vi "MecaOdometry_Update.vi"(9 "WheelPosition":T1 {"RearRight" format="%19.3f"; "RearLeft" format="%19.3f"; "FrontRight" format="%19.3f"; "FrontLeft" format="%19.3f"}, 10 "GyroAngle":T5={"VALUE"=0.0, "COS"=1.0, "SIN"=0.0} {"SIN" format="%13.4f"; "COS" format="%13.4f"; "VALUE" format="%13.4f"}, 11 "in MECA_DRIVE_ODOMETRY":T2={"POSE"={"TRANSLATION"={"X"=0.0, "Y"=0.0}, "ROTATION"={"VALUE"=0.0, "COS"=1.0, "SIN"=0.0}}, "GyroOffset"={"VALUE"=0.0, "COS"=0.0, "SIN"=0.0}, "PreviousAngle"={"VALUE"=0.0, "COS"=0.0, "SIN"=0.0}, "Kinematics"={"FrontLeft"={"X"=0.0, "Y"=0.0}, "FrontRight"={"X"=0.0, "Y"=0.0}, "RearLeft"={"X"=0.0, "Y"=0.0}, "RearRight"={"X"=0.0, "Y"=0.0}, "InverseKinematics"=[[0.0, 1.0, -1.0, 0.0], [0.0, 1.0, 1.0, 0.0], [0.0, 1.0, 1.0, 0.0], [0.0, 1.0, -1.0, 0.0]], "ForwardKinematics"=[[0.0, 1.0, -1.0, 0.0], [0.0, 1.0, 1.0, 0.0], [0.0, 1.0, 1.0, 0.0], [0.0, 1.0, -1.0, 0.0]], "PrevCoR"={"X"=0.0, "Y"=0.0}}, "PreviousWheelPositions"={"FrontLeft"=0.0, "FrontRight"=0.0, "RearLeft"=0.0, "RearRight"=0.0, "P"=FALSE}} {"PreviousWheelPositions"."RearRight" format="%19.3f"; "PreviousWheelPositions"."RearLeft" format="%19.3f"; "PreviousWheelPositions"."FrontRight" format="%19.3f"; "PreviousWheelPositions"."FrontLeft" format="%19.3f"; "Kinematics"."PrevCoR"."Y" format="%14.3f"; "Kinematics"."PrevCoR"."X" format="%14.3f"; "Kinematics"."RearRight"."Y" format="%14.3f"; "Kinematics"."RearRight"."X" format="%14.3f"; "Kinematics"."RearLeft"."Y" format="%14.3f"; "Kinematics"."RearLeft"."X" format="%14.3f"; "Kinematics"."FrontRight"."Y" format="%14.3f"; "Kinematics"."FrontRight"."X" format="%14.3f"; "Kinematics"."FrontLeft"."Y" format="%14.3f"; "Kinematics"."FrontLeft"."X" format="%14.3f"; "PreviousAngle"."SIN" format="%13.4f"; "PreviousAngle"."COS" format="%13.4f"; "PreviousAngle"."VALUE" format="%13.4f"; "GyroOffset"."SIN" format="%13.4f"; "GyroOffset"."COS" format="%13.4f"; "GyroOffset"."VALUE" format="%13.4f"; "POSE"."ROTATION"."SIN" format="%13.4f"; "POSE"."ROTATION"."COS" format="%13.4f"; "POSE"."ROTATION"."VALUE" format="%13.4f"; "POSE"."TRANSLATION"."Y" format="%14.3f"; "POSE"."TRANSLATION"."X" format="%14.3f"}) -> (1 "POSE":T3={"TRANSLATION"={"X"=0.0, "Y"=0.0}, "ROTATION"={"VALUE"=0.0, "COS"=1.0, "SIN"=0.0}} {"ROTATION"."SIN" format="%13.4f"; "ROTATION"."COS" format="%13.4f"; "ROTATION"."VALUE" format="%13.4f"; "TRANSLATION"."Y" format="%14.3f"; "TRANSLATION"."X" format="%14.3f"}, 3 "out MECA_DRIVE_ODOMETRY":T2={"POSE"={"TRANSLATION"={"X"=0.0, "Y"=0.0}, "ROTATION"={"VALUE"=0.0, "COS"=1.0, "SIN"=0.0}}, "GyroOffset"={"VALUE"=0.0, "COS"=0.0, "SIN"=0.0}, "PreviousAngle"={"VALUE"=0.0, "COS"=0.0, "SIN"=0.0}, "Kinematics"={"FrontLeft"={"X"=0.0, "Y"=0.0}, "FrontRight"={"X"=0.0, "Y"=0.0}, "RearLeft"={"X"=0.0, "Y"=0.0}, "RearRight"={"X"=0.0, "Y"=0.0}, "InverseKinematics"=[[0.0, 1.0, -1.0, 0.0], [0.0, 1.0, 1.0, 0.0], [0.0, 1.0, 1.0, 0.0], [0.0, 1.0, -1.0, 0.0]], "ForwardKinematics"=[[0.0, 1.0, -1.0, 0.0], [0.0, 1.0, 1.0, 0.0], [0.0, 1.0, 1.0, 0.0], [0.0, 1.0, -1.0, 0.0]], "PrevCoR"={"X"=0.0, "Y"=0.0}}, "PreviousWheelPositions"={"FrontLeft"=0.0, "FrontRight"=0.0, "RearLeft"=0.0, "RearRight"=0.0, "P"=FALSE}} {"PreviousWheelPositions"."RearRight" format="%19.3f"; "PreviousWheelPositions"."RearLeft" format="%19.3f"; "PreviousWheelPositions"."FrontRight" format="%19.3f"; "PreviousWheelPositions"."FrontLeft" format="%19.3f"; "Kinematics"."PrevCoR"."Y" format="%14.3f"; "Kinematics"."PrevCoR"."X" format="%14.3f"; "Kinematics"."RearRight"."Y" format="%14.3f"; "Kinematics"."RearRight"."X" format="%14.3f"; "Kinematics"."RearLeft"."Y" format="%14.3f"; "Kinematics"."RearLeft"."X" format="%14.3f"; "Kinematics"."FrontRight"."Y" format="%14.3f"; "Kinematics"."FrontRight"."X" format="%14.3f"; "Kinematics"."FrontLeft"."Y" format="%14.3f"; "Kinematics"."FrontLeft"."X" format="%14.3f"; "PreviousAngle"."SIN" format="%13.4f"; "PreviousAngle"."COS" format="%13.4f"; "PreviousAngle"."VALUE" format="%13.4f"; "GyroOffset"."SIN" format="%13.4f"; "GyroOffset"."COS" format="%13.4f"; "GyroOffset"."VALUE" format="%13.4f"; "POSE"."ROTATION"."SIN" format="%13.4f"; "POSE"."ROTATION"."COS" format="%13.4f"; "POSE"."ROTATION"."VALUE" format="%13.4f"; "POSE"."TRANSLATION"."Y" format="%14.3f"; "POSE"."TRANSLATION"."X" format="%14.3f"})   [LabVIEW 2019, in "Trajectory_Library.lvlib"]
doc: "Updates the robot's position on the field using forward kinematics and integration of the pose over time. This method takes in an angle parameter which is used instead of the angular rate that is calculated from forward kinematics, in addition to the current distance measurement at each wheel.\n \nParameters:\n - MecaDriveOdometry - Data structure\n - gyroAngle - The angle reported by the gyroscope.\n - wheelPositions - The distances driven by each wheel..\n\nReturns:\n - MecaDriveOdometry - Updated data structure\n - Pose - The new pose of the robot."
uses:
  Trajectory_Library.lvlib
  TypeDef/MECA_DRIVE_ODOMETRY.ctl
  TypeDef/POSE2D.ctl
  TypeDef/TRANSLATION2D.ctl
  TypeDef/ROTATION2D.ctl
  TypeDef/MECA_DRIVE_KINEMATICS.ctl
  <vilib>/Analysis/Matrix/Datatypes/RealMatrix.ctl
  TypeDef/MECA_WHEEL_POSITIONS.ctl
  VI/MecaWheelPos_Get.vi
  VI/MecaWheelPos_New.vi
  Rotation2d_RotateBy.vi
  Rotation2d_UnaryMinus.vi
  Rotation2d_CreateXY.vi
  Rotation2d_CreateAngle.vi
  Util_CalcDist.vi
  <vilib>/Analysis/Matrix/NI_Matrix.lvlib
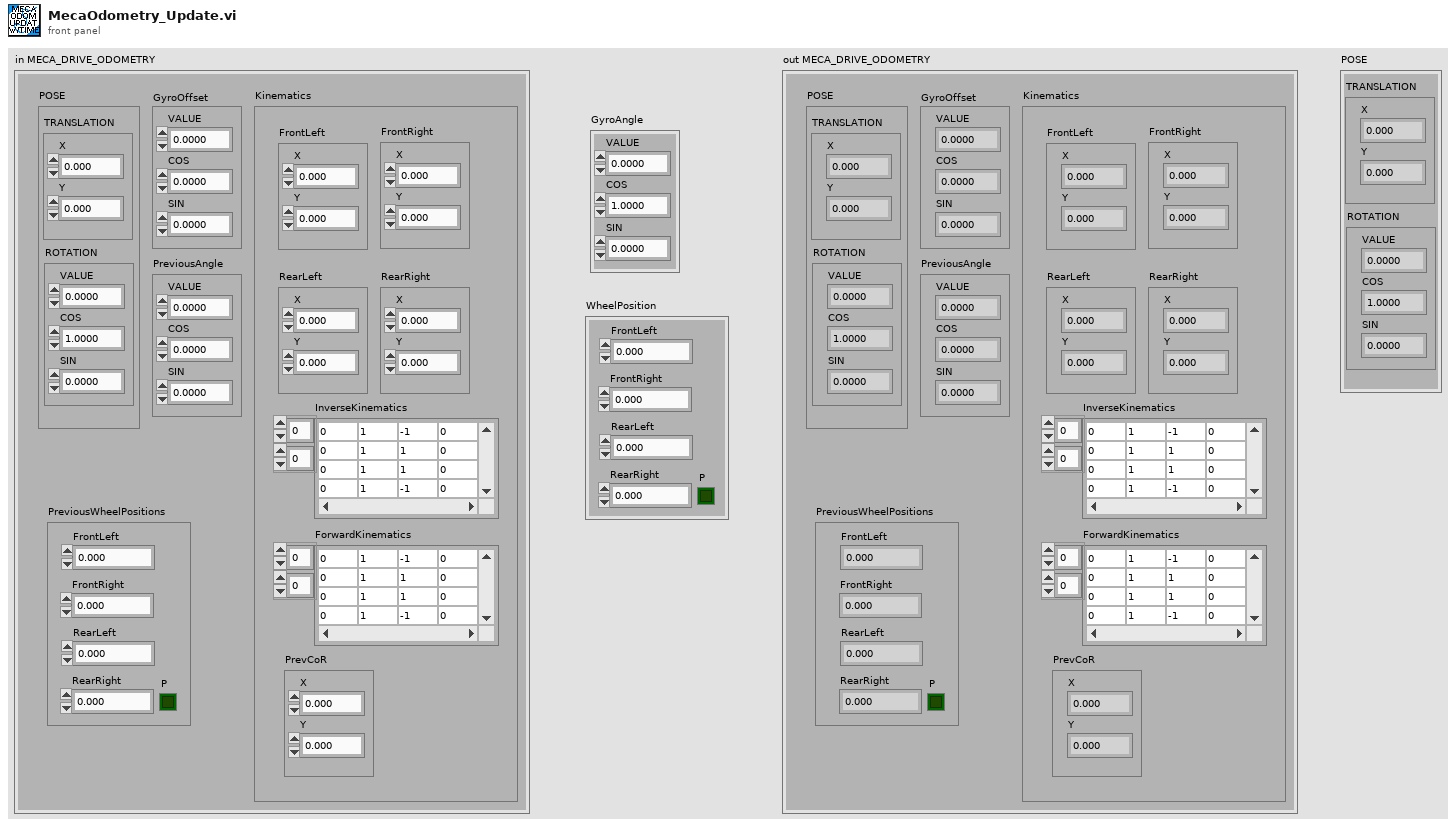
[diagram p1: front panel]
types:
  T1 = typedef "Trajectory_Library.lvlib/MECA_WHEEL_POSITIONS.ctl" = cluster{"FrontLeft":dbl, "FrontRight":dbl, "RearLeft":dbl, "RearRight":dbl, "P":bool}
  T2 = typedef "Trajectory_Library.lvlib/MECA_DRIVE_ODOMETRY.ctl" = cluster{"POSE":T3, "GyroOffset":T5, "PreviousAngle":T5, "Kinematics":T6, "PreviousWheelPositions":T1}
  T3 = typedef "Trajectory_Library.lvlib/POSE2D.ctl" = cluster{"TRANSLATION":T4, "ROTATION":T5}
  T4 = typedef "Trajectory_Library.lvlib/TRANSLATION2D.ctl" = cluster{"X":dbl, "Y":dbl}
  T5 = typedef "Trajectory_Library.lvlib/ROTATION2D.ctl" = cluster{"VALUE":dbl, "COS":dbl, "SIN":dbl}
  T6 = typedef "Trajectory_Library.lvlib/MECA_DRIVE_KINEMATICS.ctl" = cluster{"FrontLeft":T4, "FrontRight":T4, "RearLeft":T4, "RearRight":T4, "InverseKinematics":T7, "ForwardKinematics":T7, "PrevCoR":T4}
  T7 = typedef "NI_Matrix.lvlib/RealMatrix.ctl" = dbl[][]
  T8 = typedef "Trajectory_Library.lvlib/TWIST2D.ctl" = cluster{"dX":dbl, "dY":dbl, "dTHETA":dbl}
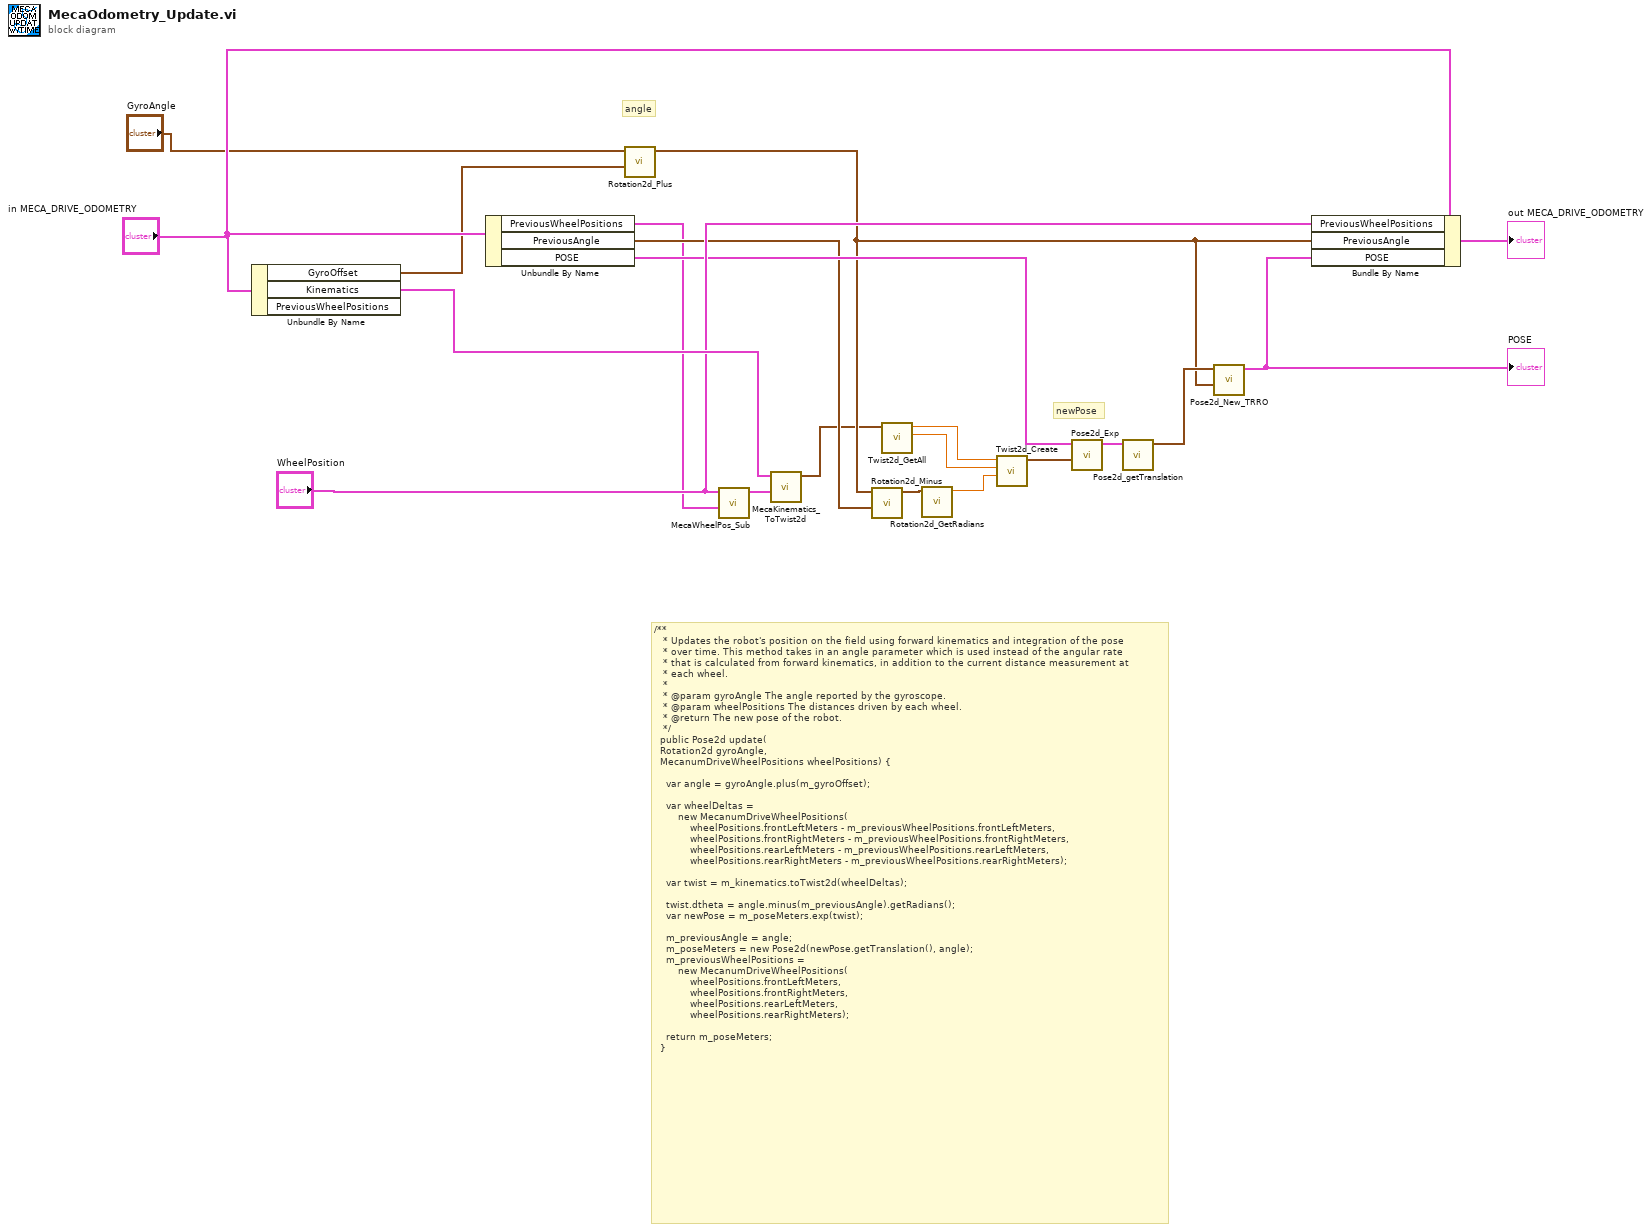
[diagram p0: block diagram]
diagram:
  # "angle"
  # "newPose"
  # "/**\n   * Updates the robot's position on the field using forward kinematics and integration of the pose\n   * over time. This method takes in an angle parameter which is used instead of the angular rate\n   * that is calculated from forward kinematics, in addition to the current distance measurement at\n   * each wheel.\n   *\n   * @param gyroAngle The angle reported by the gyroscope.\n   * @param wheelPositions The distances driven by each wheel.\n   * @return The new pose of the robot.\n   */\n  public Pose2d update(\n\t\tRotation2d gyroAngle, \n\t\tMecanumDriveWheelPositions wheelPositions) {\n\n    var angle = gyroAngle.plus(m_gyroOffset);\n\n    var wheelDeltas =\n        new MecanumDriveWheelPositions(\n            wheelPositions.frontLeftMeters - m_previousWheelPositions.frontLeftMeters,\n            wheelPositions.frontRightMeters - m_previousWheelPositions.frontRightMeters,\n            wheelPositions.rearLeftMeters - m_previousWheelPositions.rearLeftMeters,\n            wheelPositions.rearRightMeters - m_previousWheelPositions.rearRightMeters);\n\n    var twist = m_kinematics.toTwist2d(wheelDeltas);\n\n    twist.dtheta = angle.minus(m_previousAngle).getRadians();\n    var newPose = m_poseMeters.exp(twist);\n\n    m_previousAngle = angle;\n    m_poseMeters = new Pose2d(newPose.getTranslation(), angle);\n    m_previousWheelPositions =\n        new MecanumDriveWheelPositions(\n            wheelPositions.frontLeftMeters,\n            wheelPositions.frontRightMeters,\n            wheelPositions.rearLeftMeters,\n            wheelPositions.rearRightMeters);\n\n    return m_poseMeters;\n  }"
  n1 = Unbundle By Name("in MECA_DRIVE_ODOMETRY") -> ("GyroOffset"=w15:T5, "Kinematics"=w17:T6)  [unwired: 1 out]
  n2 = Unbundle By Name("in MECA_DRIVE_ODOMETRY") -> ("PreviousWheelPositions"=w3:T1, "PreviousAngle"=w11:T5, "POSE"=w12:T3)
  n3 = call "Rotation2d_Plus.vi"("other ROTATION"=w15, "in ROTATION"="GyroAngle") -> ("out ROTATION"=w2:T5)  [unwired: 9 in]
  n4 = call "MecaWheelPos_Sub.vi"("In MECA_WHEEL_POSITIONS 2"=w3, "In MECA_WHEEL_POSITIONS 1"="WheelPosition") -> ("MECA_WHEEL_POSITIONS"=w4:T1)  [unwired: 9 in]
  n5 = call "MecaKinematics_ToTwist2d.vi"("Wheel Deltat Positions"=w4, "in MECA_DRIVE_KINEMATICS"=w17) -> ("Twist2d"=w1:T8)  [unwired: 9 in]
  n6 = call "Rotation2d_Minus.vi"("other ROTATION"=w11, "in ROTATION"=w2) -> ("out ROTATION"=w10:T5)  [unwired: 9 in]
  n7 = call "Twist2d_GetAll.vi"("TWIST"=w1) -> ("dY"=w5:dbl, "dX"=w6:dbl)  [unwired: 8 in, 1 out]
  n8 = call "Rotation2d_GetRadians.vi"("in ROTATION"=w10) -> ("AngleRadians"=w9:dbl)  [unwired: 10 in]
  n9 = call "Twist2d_Create.vi"("dTHETA"=w9, "dY"=w5, "dX"=w6) -> ("TWIST"=w13:T8)  [unwired: 8 in]
  n10 = call "Pose2d_Exp.vi"("TWIST"=w13, "POSE"=w12) -> ("UpdatedPose"=w8:T3)  [unwired: 9 in]
  n11 = call "Pose2d_getTranslation.vi"("in POSE"=w8) -> ("outTRANSLATION"=w7:T4)  [unwired: 10 in]
  n12 = call "Pose2d_New_TRRO.vi"("ROTATION"=w2, "TRANSLATION"=w7) -> ("outPOSE"=w20:T3)  [unwired: 9 in]
  "POSE" <- w20
  n13 = Bundle By Name(cluster="in MECA_DRIVE_ODOMETRY", "PreviousWheelPositions"="WheelPosition", "PreviousAngle"=w2, "POSE"=w20) -> (→"out MECA_DRIVE_ODOMETRY":T2)
